vi "UE_Inclusive_Range.vi"(3 "maximum":dbl, 4 "minimum":dbl, 5 "value":dbl) -> (2 "in_range":bool)   [LabVIEW 2026]
doc: "INTENT: Evaluate a closed engineering range with both boundaries included. INPUTS: value (double), minimum (double), maximum (double). OUTPUTS: in_range (bool). DESIGN CONSTRAINT: Caller validates minimum <= maximum and quality before invocation. REQUIREMENTS: SRS-F-005. No physical hardware side effects. Acceptance requires native LabVIEW compilation and behavioral testing."
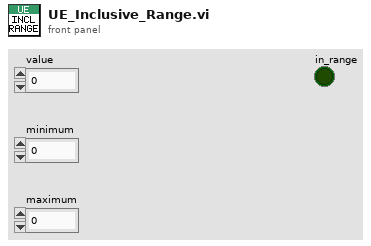
[diagram p1: front panel]
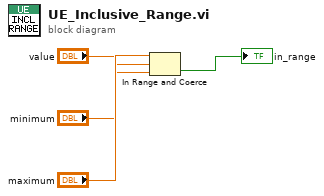
[diagram p0: block diagram]
diagram:
  n1 = In Range and Coerce(upper limit="maximum", x="value", lower limit="minimum") -> (In Range?=→"in_range":bool)  [unwired: 1 out]
